vi "Script - get FrameNames.vi"(8 "error in":errorcluster, 11 "StructRef":refnum<vi>) -> (0 "error out":errorcluster, 1 "Visible Frame Index":u32, 2 "Visible Frame Name":string, 3 "Frame Names":string[](array[string]), 4 "Visible Frame":refnum<vi>, 5 "Frames[]":refnum<vi>[](array[refnum]))   [LabVIEW 2020]
uses:
  <userlib>/_OpenG.lib/string/string.llb/Trim Whitespace (String Array)__ogtk.vi
  <userlib>/_OpenG.lib/string/string.llb/openg_string.lvlib
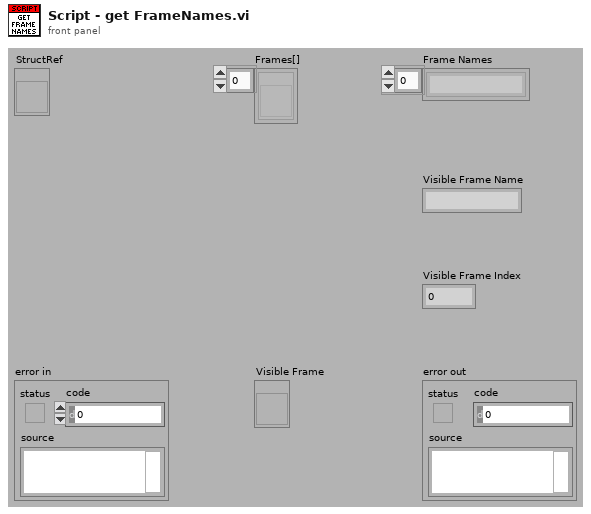
[diagram p1: front panel]
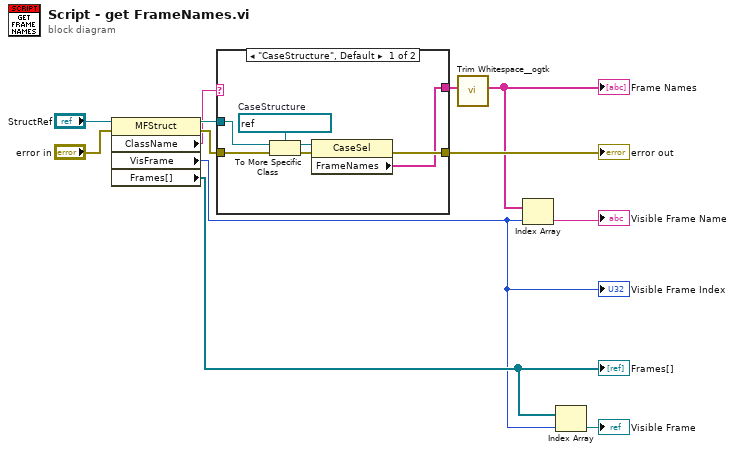
[diagram p0: block diagram]
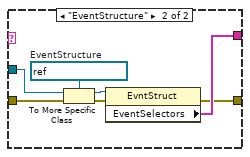
[diagram p2: hidden frame]
diagram:
  n1 = property class="MFStruct"(reference="StructRef", error in="error in") -> (reference out=w10:refnum<vi>, error out=w8:errorcluster, "ClassName"=w7:string, "VisFrame"=w3:u32, "Frames[]"=w4:refnum<vi>[])
  "Visible Frame Index" <- w3
  "Frames[]" <- w4
  n2 = case shown="\"CaseStructure\", Default" w7 {
    tunnel: w10 -> [w15 w25]
    tunnel: [w19 w21] -> w11
    tunnel: w8 -> [w18 w26]
    tunnel: [w13 w22] -> w1
    frame "CaseStructure", Default {
      w14 = refnum<vi> refnum  # CaseStructure
      n3 = To More Specific Class(target class=w14, reference=w15, error in=w18) -> (specific class reference=w16:refnum<vi>, error out=w17:errorcluster)
      n4 = property class="CaseSel"(reference=w16, error in=w17) -> (error out=w19:errorcluster, "FrameNames"=w13:string[])  [unwired: 1 out]
    }
    frame "EventStructure" {
      w24 = refnum<vi> refnum  # EventStructure
      n5 = To More Specific Class(target class=w24, reference=w25, error in=w26) -> (specific class reference=w23:refnum<vi>, error out=w20:errorcluster)
      n6 = property class="EvntStruct"(reference=w23, error in=w20) -> (error out=w21:errorcluster, "EventSelectors"=w22:string[])  [unwired: 1 out]
    }
  }
  "error out" <- w11
  n7 = call-poly <userlib>:"Trim Whitespace__ogtk.vi"("String in"=w1) -> ("String out"=w6:string[])  [unwired: 6 in]
  "Frame Names" <- w6
  n8 = Index Array(array=w6, index=w3) -> (element=→"Visible Frame Name":string)
  n9 = Index Array(array=w4, index=w3) -> (element=→"Visible Frame":refnum<vi>)
